vi "Construct.vi"(8 "error in":errorcluster, 10 "coupling mode":u32(ring) items=["API429_CHANNEL_COUPLING_EXT", "API429_CHANNEL_COUPLING_DUAL", "API429_CHANNEL_COUPLING_INT"], 11 "pxi slot":u8) -> (0 "error out":errorcluster, 3 "Shared Resources out":refnum<class "Shared Resources.lvclass">)   [LabVIEW 2020, in "AIM ARINC 429 Engine.lvlib" / "Implementation.lvlib" / "Shared Resources.lvclass"]
uses:
  Shared Resources.lvclass
  Shared Resources.lvclass/Shared Resources.ctl
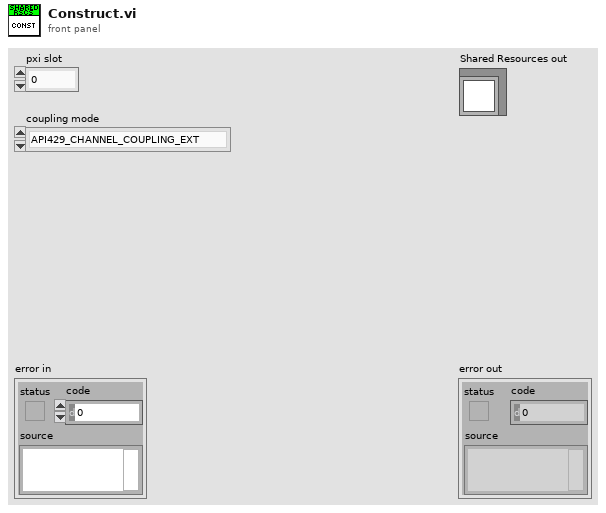
[diagram p1: front panel]
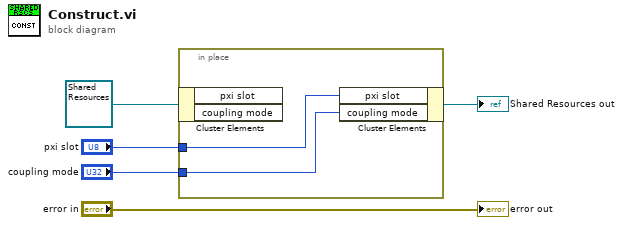
[diagram p0: block diagram]
diagram:
  n1 = in-place {
    in-place-border: "pxi slot" -> [w7]
    in-place-border: "coupling mode" -> [w6]
    n2 = in-place-cluster #1(refnum<class "Shared Resources.lvclass"> refnum ("Communication Bus Template Interfaces:Implementation.lvlib:Shared Resources.lvclass")) -> ()  [unwired: 2 out]
    n3 = in-place-cluster #1("pxi slot"=w7, "coupling mode"=w6) -> (→"Shared Resources out":refnum<class "Shared Resources.lvclass">)
  }
  "error out" <- "error in"
